vi "Create DAQmx Channels.vi"(8 "error in (no error)":errorcluster, 11 "Task In":refnum<class "Task Config.lvclass">) -> (0 "error out":errorcluster, 2 "DAQmxChannels":refnum<class "DAQmxChannel.lvclass">[](array[class]), 3 "Task":refnum<class "Task Config.lvclass">)   [LabVIEW 2020, in "VolatusDAQConfig.lvlib"]
uses:
  VolatusDAQConfig.lvlib
  VolatusConfig/Task/Task Config.lvclass
  C:/dev/lv20CE/relink/lv-volatus/VolatusConfig/VolatusConfigElement/VolatusConfigElement.lvclass
  DAQmxChannel/DAQmxChannel.lvclass
  VolatusConfig/Meta Type.ctl
  VolatusConfig/VolatusConfigElement/VolatusConfigElement.lvclass/VolatusConfigElement.ctl
  DAQmxVoltageChannel/VoltageInChannel.lvclass
  C:/dev/lv20CE/relink/lv-volatus/VolatusDAQConfig/DAQmxChannel/DAQmxChannel.lvclass
  VoltageOutChannel/VoltageOutChannel.lvclass
  CurrentOutChannel/CurrentOutChannel.lvclass
  DAQmxThermocoupleChannel/TCChannel.lvclass
  RTDChannel/RTDChannel.lvclass
  IEPEChannel/IEPEChannel.lvclass
  DigitalOutChannel/DigitalOutChannel.lvclass
  DigitalInChannel/DigitalInChannel.lvclass
  BridgeChannel/BridgeChannel.lvclass
  VolatusConfig/VolatusConfigElement/Element.vi
  lv-cdm/CDM-Config/Config Lookup/Match Meta.vi
  lv-cdm/CDM-Config/Config Element/Owner.vi
  lv-cdm/CDM-Config/Config Manager/Lookup Descendant.vi
  lv-cdm/CDM-Config/Config Filter/Config Lookup.lvclass
  VolatusConfig/VolatusConfigElement/VolatusConfigElement.lvclass
  VolatusConfig/VolatusConfig.lvlib
  lv-cdm/CDM-Config/Config Element/Config Element.lvclass
  C:/dev/lv20CE/relink/lv-volatus/VolatusConfig/Channel/Channel Config.lvclass
  CurrentInChannel/CurrentInChannel.lvclass
  C:/dev/lv20CE/relink/lv-volatus/VolatusDAQConfig/DAQmxVoltageChannel/VoltageInChannel.lvclass
  C:/dev/lv20CE/relink/lv-volatus/VolatusDAQConfig/VoltageOutChannel/VoltageOutChannel.lvclass
  C:/dev/lv20CE/relink/lv-volatus/VolatusDAQConfig/CurrentInChannel/CurrentInChannel.lvclass
  C:/dev/lv20CE/relink/lv-volatus/VolatusDAQConfig/CurrentOutChannel/CurrentOutChannel.lvclass
  C:/dev/lv20CE/relink/lv-volatus/VolatusDAQConfig/DAQmxThermocoupleChannel/TCChannel.lvclass
  C:/dev/lv20CE/relink/lv-volatus/VolatusDAQConfig/RTDChannel/RTDChannel.lvclass
  C:/dev/lv20CE/relink/lv-volatus/VolatusDAQConfig/IEPEChannel/IEPEChannel.lvclass
  C:/dev/lv20CE/relink/lv-volatus/VolatusDAQConfig/DigitalOutChannel/DigitalOutChannel.lvclass
  C:/dev/lv20CE/relink/lv-volatus/VolatusDAQConfig/DigitalInChannel/DigitalInChannel.lvclass
  C:/dev/lv20CE/relink/lv-volatus/VolatusDAQConfig/BridgeChannel/BridgeChannel.lvclass
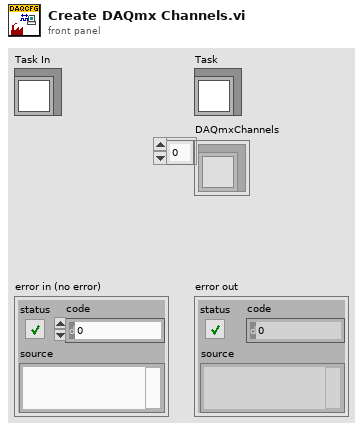
[diagram p1: front panel]
types:
  T1 = typedef "VolatusConfig.lvlib/Meta Type.ctl" = enum16{"UNKNOWN", "VL_System", "VL_Cluster", "VL_Node", "VL_Task", "VL_Group", "VL_Channel", "VL_Task_List", "VL_Scaling", "VL_Sensor", "VL_Sensor_List", "VL_Scale"}
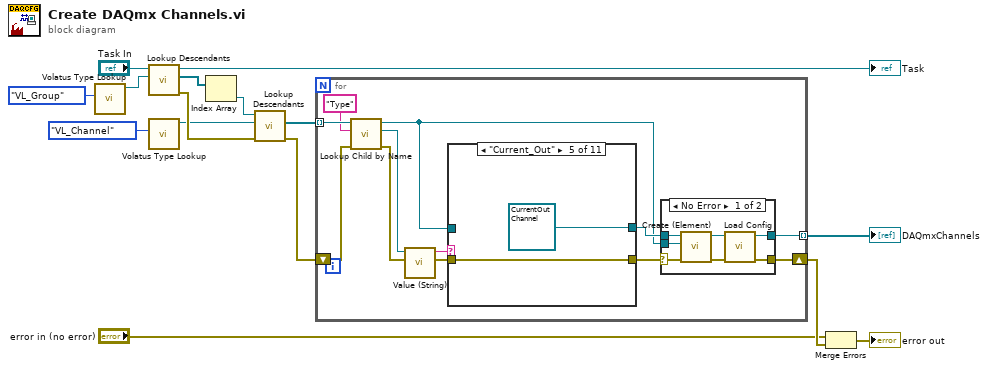
[diagram p0: block diagram]
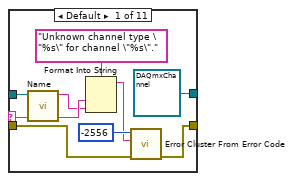
[diagram p3: hidden frame]
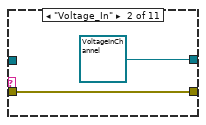
[diagram p4: hidden frame]
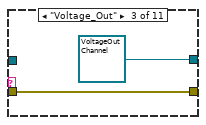
[diagram p5: hidden frame]
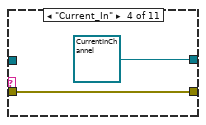
[diagram p6: hidden frame]
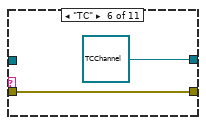
[diagram p7: hidden frame]
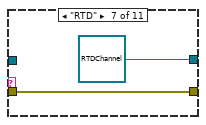
[diagram p8: hidden frame]
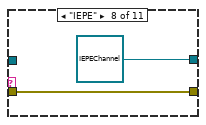
[diagram p9: hidden frame]
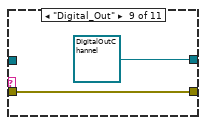
[diagram p10: hidden frame]
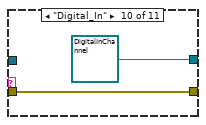
[diagram p11: hidden frame]
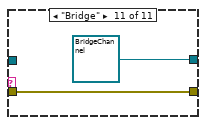
[diagram p12: hidden frame]
diagram:
  n1 = call "Volatus Type Lookup.vi"("Meta Type"=Meta_Type."VL_Group") -> ("Config Lookup out"=w14:refnum<class "Config Lookup.lvclass">)  [unwired: 9 in, 1 out]
  n2 = call "Lookup Descendants.vi"("Lookup"=w14, "VolatusConfigElement in"="Task In") -> ("error out"=w9:errorcluster, "Descendants"=w12:refnum<class "Config Element.lvclass">[], "VolatusConfigElement out"=→"Task":refnum<class "Task Config.lvclass">)  [unwired: 7 in]
  n3 = call "Volatus Type Lookup.vi"("Meta Type"=Meta_Type."VL_Channel") -> ("Config Lookup out"=w8:refnum<class "Config Lookup.lvclass">)  [unwired: 9 in, 1 out]
  n4 = Index Array(array=w12) -> (element=w11:refnum<class "Config Element.lvclass">)  [unwired: 1 in]
  n5 = call "Lookup Descendants.vi"("error in (no error)"=w9, "Lookup"=w8, "Config Element in"=w11) -> ("error out"=w6:errorcluster, "Descendants"=w7:refnum<class "Config Element.lvclass">[])  [unwired: 6 in, 1 out]
  n6 = for {
    tunnel: w7 -> [w26] mode=indexing
    shift-right: [w21] -> w3
    shift-left: w6 -> [w27]
    tunnel: [w20] -> w5 mode=indexing
    n7 = call "Lookup Child by Name.vi"("error in (no error)"=w27, "Name"="Type", "Config Element in"=w26) -> ("error out"=w24:errorcluster, "Child"=w17:refnum<class "Config Element.lvclass">, "Config Element out"=w16:refnum<class "Config Element.lvclass">)  [unwired: 5 in, 1 out]
    n8 = call "Value (String).vi"("error in (no error)"=w24, "Config Element in"=w17) -> ("error out"=w22:errorcluster, "String Value"=w23:string)  [unwired: 8 in]
    n9 = case shown="\"Current_Out\"" w23 {
      selector: w23 -> [w42 _ _ _ _ _ _ _ _ _ _]
      tunnel: w22 -> [w44 w46 w48 w50 w52 w54 w56 w58 w60 w62 w64]
      tunnel: [w38 w46 w48 w50 w52 w54 w56 w58 w60 w62 w64] -> w19
      tunnel: w16 -> [w37 _ _ _ _ _ _ _ _ _ _]
      tunnel: [refnum<class "DAQmxChannel.lvclass"> refnum ("VolatusDAQConfig:DAQmxThermocoupleChannel") refnum<class "VoltageInChannel.lvclass"> refnum ("VolatusDAQConfig:DAQmxVoltageChannel.lvclass") refnum<class "VoltageOutChannel.lvclass"> refnum ("VolatusDAQConfig:VoltageOutChannel.lvclass") refnum<class "CurrentInChannel.lvclass"> refnum ("VolatusDAQConfig:CurrentInChannel.lvclass") refnum<class "CurrentOutChannel.lvclass"> refnum ("VolatusDAQConfig:CurrentOutChannel.lvclass") refnum<class "TCChannel.lvclass"> refnum ("VolatusDAQConfig:DAQmxThermocoupleChannel") refnum<class "RTDChannel.lvclass"> refnum ("VolatusDAQConfig:RTDChannel.lvclass") refnum<class "IEPEChannel.lvclass"> refnum ("VolatusDAQConfig:IEPEChannel.lvclass") refnum<class "DigitalOutChannel.lvclass"> refnum ("VolatusDAQConfig:DigitalOutChannel.lvclass") refnum<class "DigitalInChannel.lvclass"> refnum ("VolatusDAQConfig:DigitalInChannel.lvclass") refnum<class "BridgeChannel.lvclass"> refnum ("VolatusDAQConfig:BridgeChannel.lvclass")] -> w18
      frame Default {
        n10 = call "Name.vi"("Config Element in"=w37) -> ("Name"=w39:string)  [unwired: 9 in, 1 out]
        n11 = Format Into String(format string="Unknown channel type \"%s\" for channel \"%s\".", w42, w39) -> (resulting string=w41:string)  [unwired: 2 in, 1 out]
        n12 = call <vilib>:"Error Cluster From Error Code.vi"("error in (no error)"=w44, "error message (\"\")"=w41, "error code (0)"=-2556) -> ("error out"=w38:errorcluster)  [unwired: 6 in]
      }
      frame "Voltage_In" {
      }
      frame "Voltage_Out" {
      }
      frame "Current_In" {
      }
      frame "Current_Out" {
      }
      frame "TC" {
      }
      frame "RTD" {
      }
      frame "IEPE" {
      }
      frame "Digital_Out" {
      }
      frame "Digital_In" {
      }
      frame "Bridge" {
      }
    }
    n13 = case shown="No Error" w19 {
      selector: w19 -> [w31 w35]
      tunnel: [w34 w35] -> w21
      tunnel: [w33 _] -> w20
      tunnel: w18 -> [w30 _]
      tunnel: w16 -> [w29 _]
      frame No Error {
        n14 = call "Create (Element).vi"("error in (no error)"=w31, "Element"=w29, "VolatusConfigElement in"=w30) -> ("error out"=w32:errorcluster, "VolatusConfigElement out"=w28:refnum<class "DAQmxChannel.lvclass">)  [unwired: 7 in]
        n15 = call-dynamic "Load Config.vi"("error in (no error)"=w32, "DAQmxChannel in"=w28) -> ("error out"=w34:errorcluster, "DAQmxChannel out"=w33:refnum<class "DAQmxChannel.lvclass">)  [unwired: 8 in]
      }
      frame Error {
      }
    }
  }
  "DAQmxChannels" <- w5
  n16 = Merge Errors("error in (no error)", w3) -> (→"error out":errorcluster)
